vi "lvmcp_bunnames.vi"() -> ()   [LabVIEW 2015]
panel:
  in  "names":string[](array[string])
  out "error out":errorcluster
  in  "count":i32
  in  "reference":refnum<vi>
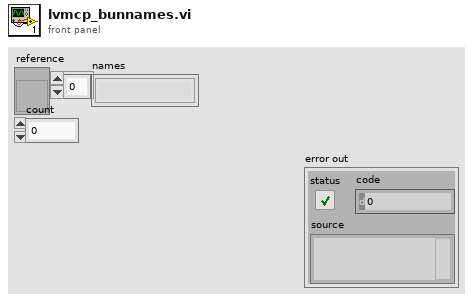
[diagram p1: front panel]
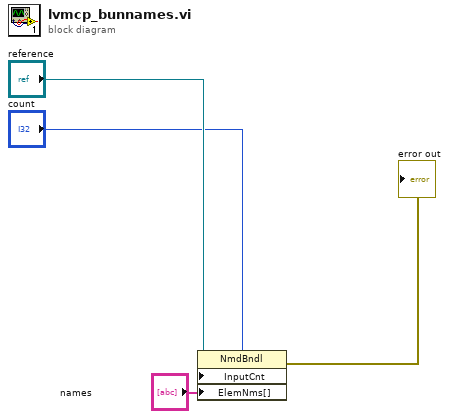
[diagram p0: block diagram]
diagram:
  n1 = property class="NmdBndl"(reference="reference", "InputCnt"="count", "ElemNms[]"="names") -> (error out=→"error out":errorcluster)  [unwired: 1 in, 1 out]
